vi "DFT_Spectra UI.vi"(10 "averages completed":dbl, 11 "Spectrum Data":refnum<class "Data.lvclass">) -> ()   [LabVIEW 2024, in "DFT_Spectra.lvlib" / "DFT_Spectra.lvclass"]
uses:
  DFT_Spectra.lvclass
  <vilib>/addons/_XControls/Spectrum with Cursors/Spectrum with Cursors.xctl
  <vilib>/addons/_NISVFA/_Shared subVIs/Data Objects/Data/Data.lvclass
  DFT_Spectra.lvclass/DFT_Spectra.ctl
panel:
  out "Averages completed":dbl format="%#_10g"
  out "Spectrum with Cursors":refnum<class "Data.lvclass">(xcontrol)
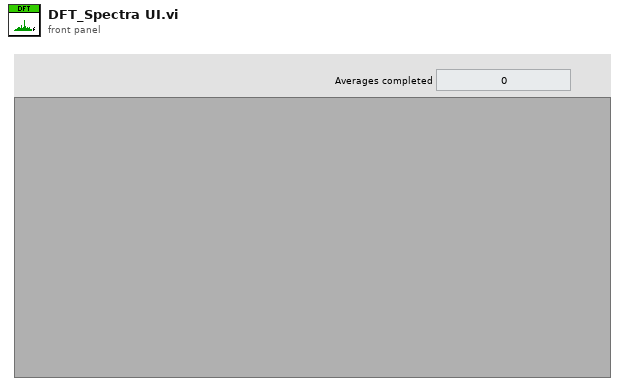
[diagram p1: front panel]
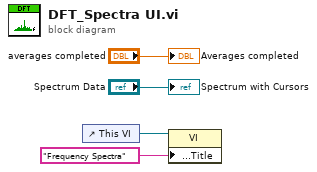
[diagram p0: block diagram]
diagram:
  n1 = control-ref of="This VI"() -> (w2:refnum<vi>)
  n2 = property class="VI"(reference=w2, "Front Panel.Title"="Frequency Spectra" ("Front Panel Window:Title")) -> ()  [unwired: 1 in, 2 out]
  "Averages completed" <- "averages completed"
  "Spectrum with Cursors" <- "Spectrum Data"
